vi "VIH Constant - Icon 32x32 - Unknown.vi"() -> (3 "image data":T1={"image type"=0, "image depth"=24, "image"=array[3072 elements], "mask"=[], "colors"=[], "Rectangle"={"left"=0, "top"=0, "right"=32, "bottom"=32}})   [LabVIEW 2014]
doc: "::: VI Helpeks :::\nCopyright (c) 2000-2026 Konstantin Shifershteyn. All rights reserved."
uses:
  <vilib>/picture/picture.llb/imagedata.ctl
panel:
  # "VI Helpeks\nCopyright (c) 2012-2026 Konstantin Shifershteyn"
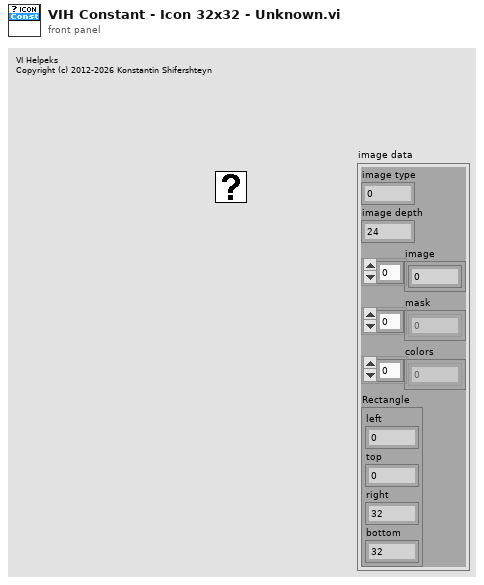
[diagram p1: front panel]
types:
  T1 = typedef "imagedata.ctl" = cluster{"image type":i32, "image depth":i32, "image":u8[], "mask":u8[], "colors":u32[], "Rectangle":cluster{"left":i16, "top":i16, "right":i16, "bottom":i16}}
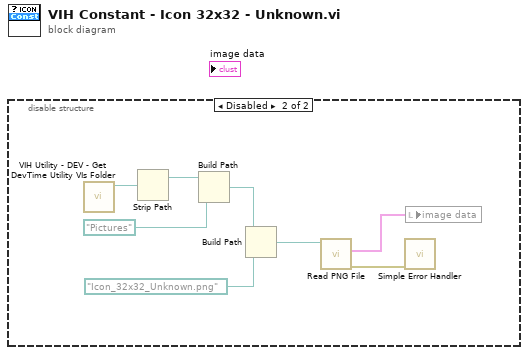
[diagram p0: block diagram]
diagram:
  n1 = disable-structure shown="Disabled" {
    frame Enabled {
    }
    frame Disabled {
      n2 = call "VIH Utility - DEV - Get DevTime Utility VIs Folder.vi"() -> ("Utility VIs Folder"=w8:path)  [unwired: 9 in, 2 out]
      n3 = Strip Path(path=w8) -> (stripped path=w7:path)  [unwired: 1 out]
      n4 = Build Path(base path=w7, name or relative path=path "Pictures") -> (appended path=w4:path)
      n5 = Build Path(base path=w4, name or relative path=path "Icon_32x32_Unknown.png") -> (appended path=w5:path)
      n6 = call <vilib>:"Read PNG File.vi"("path to PNG file"=w5) -> ("error out"=w2:errorcluster, "image data"=w1:T1)  [unwired: 8 in, 1 out]
      n7 = call <vilib>:"Simple Error Handler.vi"("error in (no error)"=w2) -> ()  [unwired: 4 in, 5 out]
      n8 = local write "image data"(w1) -> ()
    }
  }
